vi "VIH Dialog - Enum Values.vi"(8 "VI Path":path, 9 "Control ID":string, 10 "EnumValDefs in":T6[](array[typedef]), 11 "Project Tree":T1) -> (0 "OK out":bool, 2 "EnumValDefs out":T6[](array[typedef]))   [LabVIEW 2014]
doc: "::: VI Helpeks :::\nCopyright (c) 2000-2026 Konstantin Shifershteyn. All rights reserved."
uses:
  _VIH UI Controls.llb/VIH UI Control - Button - Insert HREF.ctl
  _VIH UI Controls.llb/VIH UI Control - Button - Insert Bold.ctl
  _VIH UI Controls.llb/VIH UI Control - Button - Insert Italic.ctl
  _VIH UI Controls.llb/VIH UI Control - Button - Insert Underline.ctl
  _VIH HelpGen.llb/VIH HelpGen Typedef - Cluster - Enum Value Info.ctl
  VIH Project Tree Typedef - Tree Refnum.ctl
  <vilib>/Utility/miscctls.llb/LVRowAndColumnUnsignedTypeDef.ctl
panel:
  in  "%Sort":bool caption="Sort"
  in  "%Import":bool caption="Import"
  in  "%Insert_<I>":T2 caption="Format as Italic"
  in  "%Insert_<U>":T3 caption="Format as Underline"
  in  "%Insert_<B>":T4 caption="Format as Bold"
  in  "%Insert_HREF":T5 caption="Insert Reference"
  in  "Description":string
  in  "String":string
  in  "Value":ext
  in  "%Cancel":bool caption="Cancel"
  in  "%OK":bool caption="OK"
  in  "%Remove":bool caption="Remove"
  in  "%Add":bool caption="Add"
  in  "Val List":i32[](listbox) caption="Value List"
  # "*) use Context Help for information on the controls"
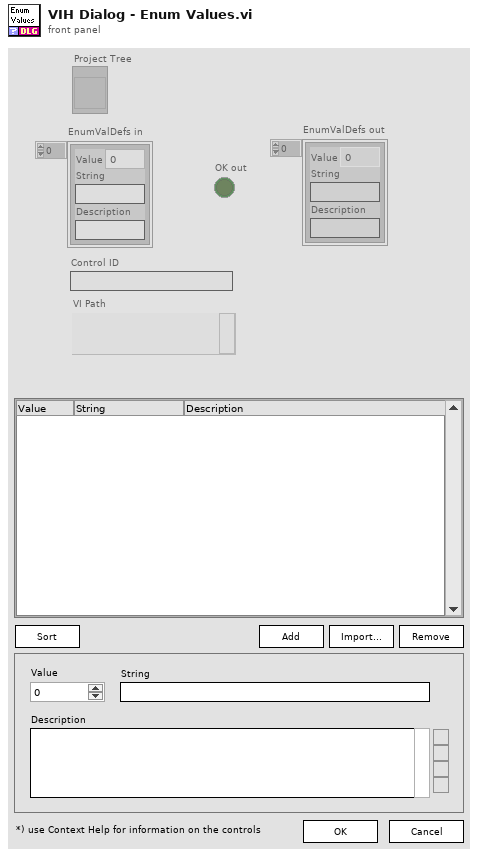
[diagram p1: front panel]
types:
  T1 = typedef "VIH Project Tree Typedef - Tree Refnum.ctl" = refnum<vi>
  T2 = typedef "VIH UI Control - Button - Insert Italic.ctl" = bool
  T3 = typedef "VIH UI Control - Button - Insert Underline.ctl" = bool
  T4 = typedef "VIH UI Control - Button - Insert Bold.ctl" = bool
  T5 = typedef "VIH UI Control - Button - Insert HREF.ctl" = bool
  T6 = typedef "VIH HelpGen Typedef - Cluster - Enum Value Info.ctl" = cluster{"Value":ext, "String":string, "Description":string}
  T7 = typedef "LVRowAndColumnUnsignedTypeDef.ctl" = cluster{"Row":u32, "Column":u32}
  T8 = typedef "lveventtype.ctl" = enum32{"Null", "Timeout", "Annotation Menu Selection", "Annotation Menu Selection?", "App Instance Close", "App Instance Close?", "Autoscale Range Change", "Bookmark Info Change", "Cell Edit", "Cell Edit?", "Cursor Grab", "Cursor Grab?", "Cursor Menu Selection", "Cursor Menu Selection?", "Cursor Move", "Cursor Release", "Data Change", "Direction Change", "Display State Change", "Drag Ended", "Drag Enter", "Drag Leave", "Drag Over", "Drag Source Update", "Drag Starting", "Drag Starting?", "Drop", "Exec State Change", "Key Down", "Key Down?", "Key Repeat", "Key Repeat?", "Key Up", "Listbox Double Click", "Menu Activation?", "Menu Selection (App)", "Menu Selection? (App)", "Menu Selection (User)", "Mouse Down", "Mouse Down?", "Mouse Enter", "Mouse Leave", "Mouse Move", "Mouse Up", "Mouse Wheel", "NI Security User Change (App)", "Pane Size", "Panel Close", "Panel Close?", "Panel Resize", "Plot Attribute Change", "Scale Range Change", "Shortcut Menu Activation?", "Shortcut Menu Selection (App)", "Shortcut Menu Selection? (App)", "Shortcut Menu Selection (User)", "Tree Double Click", "Tree Drag", "Tree Drag?", "Tree Drop", "Tree Drop?", "Tree Item Close", "Tree Item Close?", "Tree Item Open", "Tree Item Open?", "User Event", "Value Change"}
  T9 = enum8{"Enabled", "Disabled", "Disabled and Grayed Out"}
  T10 = typedef "VIH HelpGen Typedef - Cluster - Control Rule.ctl" = cluster{"CtrlID":string, "CustomRule":bool, "DscrMode":T11, "Description":string, "ClusterMembers":T12, "EnumValues":T12, "EnumValDscr":T6[], "CustomName":string}
  T11 = typedef "VIH HelpGen Typedef - Enum - Description Mode.ctl" = enum16{"Default", "Description", "Description1", "Description2", "Custom", "None"}
  T12 = typedef "VIH HelpGen Typedef - Enum - Default,Enable,Disable.ctl" = enum16{"Default", "Enable", "Disable"}
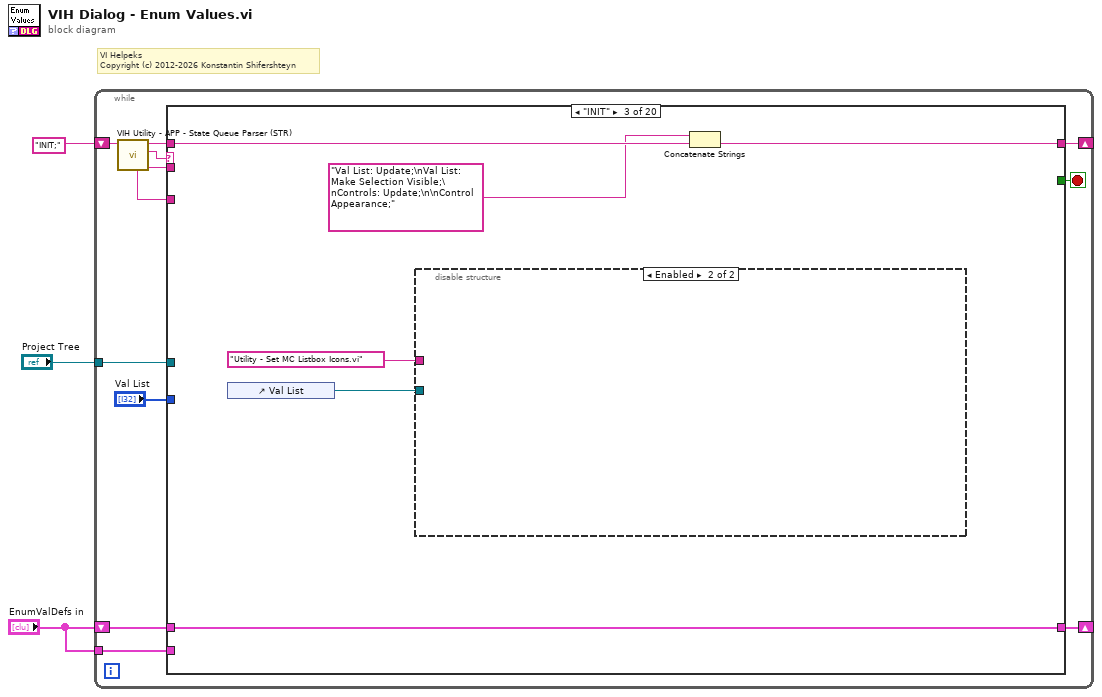
[diagram p0: block diagram]
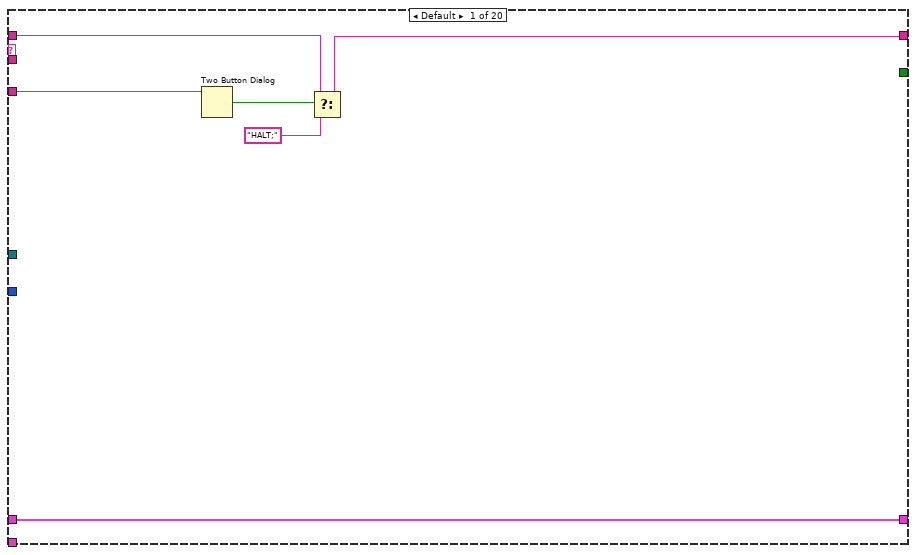
[diagram p2: hidden frame]
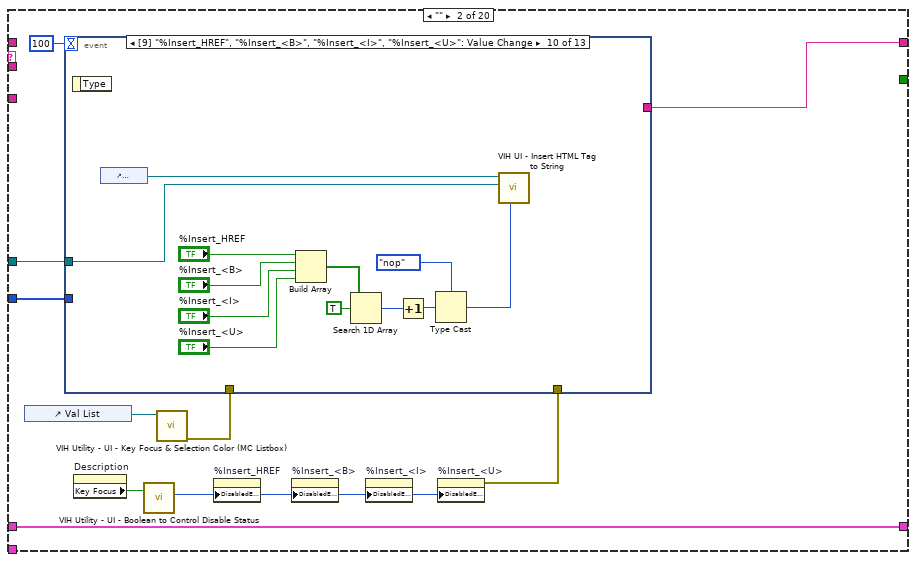
[diagram p3: hidden frame]
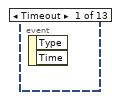
[diagram p4: hidden frame]
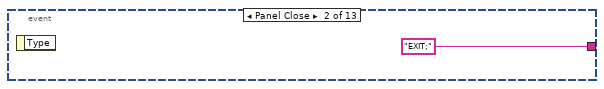
[diagram p5: hidden frame]
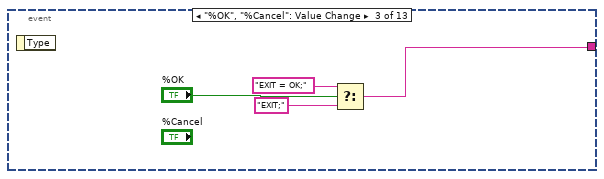
[diagram p6: hidden frame]
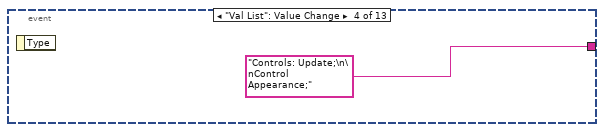
[diagram p7: hidden frame]
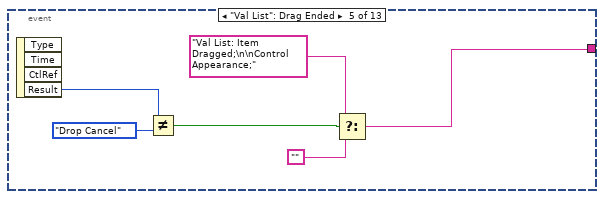
[diagram p8: hidden frame]
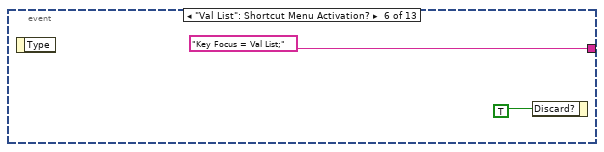
[diagram p9: hidden frame]
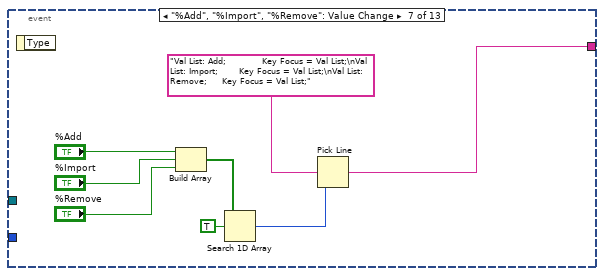
[diagram p10: hidden frame]
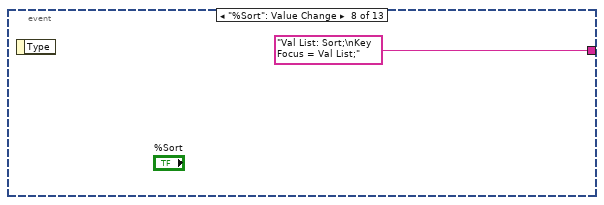
[diagram p11: hidden frame]
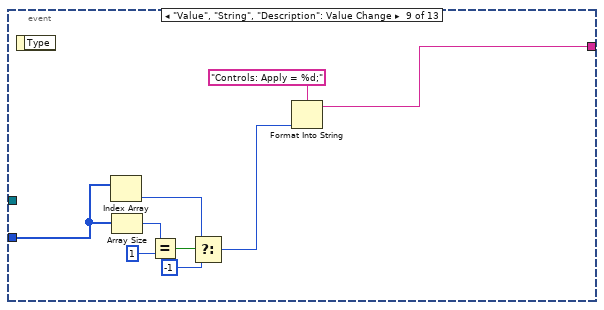
[diagram p12: hidden frame]
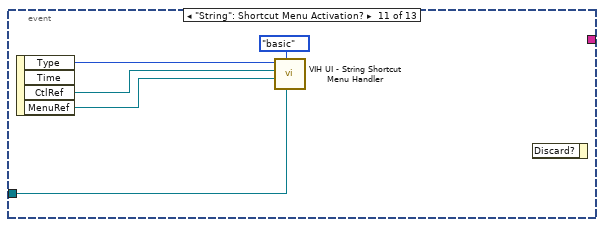
[diagram p13: hidden frame]
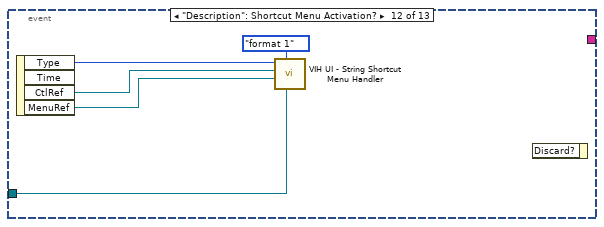
[diagram p14: hidden frame]
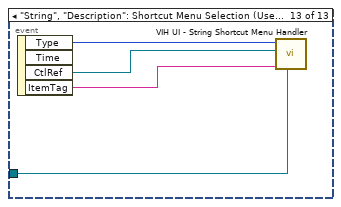
[diagram p15: hidden frame]
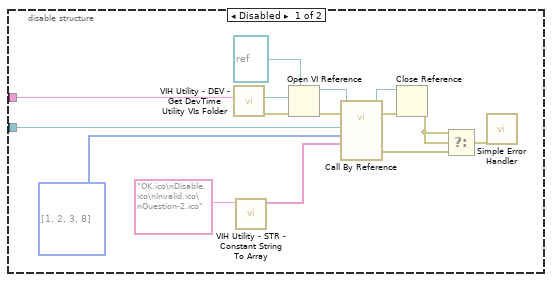
[diagram p16: hidden frame]
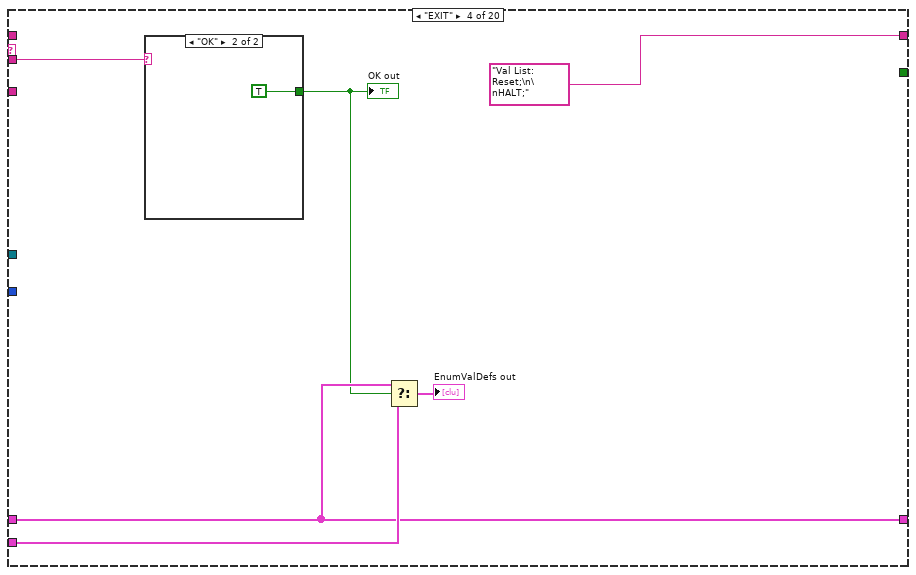
[diagram p17: hidden frame]
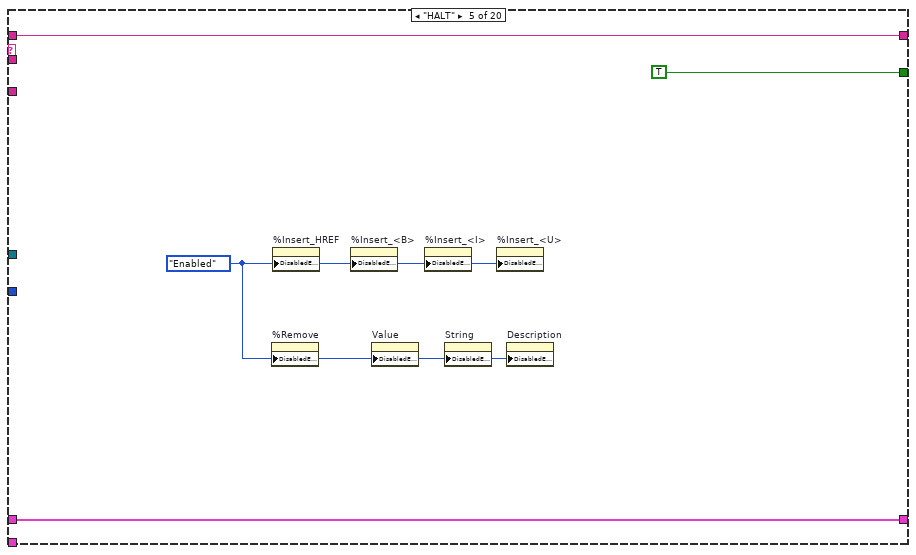
[diagram p19: hidden frame]
diagram:
  # "VI Helpeks\nCopyright (c) 2012-2026 Konstantin Shifershteyn"
  n1 = while {
    shift-right: [w11] -> _
    shift-left: "INIT;" -> [w15]
    shift-right: [w8] -> _
    shift-left: "EnumValDefs in" -> [w9]
    tunnel: "EnumValDefs in" -> [w7]
    tunnel: "Project Tree" -> [w4]
    stop <- w6 stop-if-true
    n2 = call "VIH Utility - APP - State Queue Parser (STR).vi"("input queue"=w15) -> ("state parameters"=w10:string, "state"=w14:string, "remained queue"=w12:string, "complete state specifier"=w13:string)  [unwired: 5 in]
    n3 = case shown="\"INIT\"" w14 {
      tunnel: w13 -> [w21 _ _ _ _ _ _ _ _ _ _ _ _ _ _ _ _ _ _ _]
      tunnel: w12 -> [w19 _ w95 _ w120 w122 w125 w131 w133 w139 w149 w169 w228 w250 w271 w339 w350 w354 w364 w380]
      tunnel: [w18 w30 w94 "Val List: Reset;\n\nHALT;" w120 w122 w125 w131 w133 w139 w148 w169 w228 w249 w270 w338 w345 w354 w364 w374] -> w11
      tunnel: w10 -> [_ _ _ w115 _ _ w124 _ _ _ _ _ _ _ _ _ _ _ _ w377]
      tunnel: w9 -> [w16 w31 w92 w113 w121 w123 w126 w132 w134 _ w144 w165 w229 w230 w267 w325 w347 w355 w361 w379]
      tunnel: [w16 w31 w92 w113 w121 w123 w126 w132 w134 T6[] [] ("EnumValDefs in") w143 w165 w229 w247 w268 w324 w346 w355 w361 w378] -> w8
      tunnel: w7 -> [_ _ _ w114 _ _ _ _ _ _ _ _ _ _ _ _ _ _ _ _]
      tunnel: [_ _ _ _ TRUE _ _ _ _ _ _ _ _ _ _ _ _ _ _ _] -> w6
      tunnel: "Val List" -> [_ w26 _ _ _ _ _ w130 _ _ w142 _ _ w243 _ w326 _ _ w363 _]
      tunnel: w4 -> [_ w22 _ _ _ _ _ _ _ _ _ _ _ _ w262 _ _ _ _ _]
      frame Default {
        n4 = Two Button Dialog(message=w21) -> (T button?=w20:bool)  [unwired: 2 in]
        n5 = Select(t=w19, s=w20, f="HALT;") -> (s? t:f=w18:string)
      }
      frame "" {
        n6 = control-ref of="Val List"() -> (w28:refnum<vi>)
        n7 = property on="Description" class="Str"() -> ("Key Focus"=w25:bool)  [unwired: 2 in, 2 out]
        n8 = call "VIH Utility - UI - Boolean to Control Disable Status.vi"("Status in"=w25) -> ("Control Disable if False"=w23:u8)  [unwired: 3 in, 1 out]
        n9 = call "VIH Utility - UI - Key Focus & Selection Color (MC Listbox).vi"("MCListbox Refnum"=w28) -> ("error out"=w27:errorcluster)  [unwired: 8 in, 2 out]
        n10 = property on="%Insert_HREF" class="Bool"("DisabledEnum"=w23) -> ()  [unwired: 2 in, 2 out]
        n11 = property on="%Insert_<B>" class="Bool"("DisabledEnum"=w23) -> ()  [unwired: 2 in, 2 out]
        n12 = property on="%Insert_<I>" class="Bool"("DisabledEnum"=w23) -> ()  [unwired: 2 in, 2 out]
        n13 = property on="%Insert_<U>" class="Bool"("DisabledEnum"=w23) -> (error out=w24:errorcluster)  [unwired: 2 in, 1 out]
        n14 = event shown="[9] \"%Insert_HREF\", \"%Insert_<B>\", \"%Insert_<I>\", \"%Insert_<U>\": Value Change" {
          selector: _ -> [_ _ _ _ _ _ _ _ _ _ _ _ _]
          dyn-events: _ -> [_ _ _ _ _ _ _ _ _ _ _ _ _]
          timeout: 100 -> [_ _ _ _ _ _ _ _ _ _ _ _ _]
          tunnel: [_ "EXIT;" w35 "Controls: Update;\n\nControl Appearance;" w38 "Key Focus = Val List;" w47 "Val List: Sort;\nKey Focus = Val List;" ("string") w62 _ _ _ _] -> w30
          tunnel: w27 -> [_ _ _ _ _ _ _ _ _ _ _ _ _]
          tunnel: w26 -> [_ _ _ _ _ _ _ _ w58 _ _ _ _]
          tunnel: w24 -> [_ _ _ _ _ _ _ _ _ _ _ _ _]
          tunnel: w22 -> [_ _ _ _ _ _ _ _ _ w68 w76 w81 w87]
          event Timeout {
            n15 = event-data() -> ()  [unwired: 1 in, 2 out]
          }
          event Panel Close {
            n16 = event-data() -> ()  [unwired: 1 in, 1 out]
          }
          event "%OK", "%Cancel": Value Change {
            n17 = event-data() -> ()  [unwired: 1 in, 1 out]
            n18 = Select(t="EXIT = OK;", s="%OK", f="EXIT;") -> (s? t:f=w35:string)
          }
          event "Val List": Value Change {
            n19 = event-data() -> ()  [unwired: 1 in, 1 out]
          }
          event "Val List": Drag Ended {
            n20 = event-data() -> ("Result"=w43:enum16{"Drop Cancel", "Drop Move", "Drop Copy"})  [unwired: 1 in, 3 out]
            n21 = Not Equal?(x=w43, y=enum16{"Drop Cancel", "Drop Move", "Drop Copy"}."Drop Cancel") -> (x != y?=w41:bool)
            n22 = Select(t="Val List: Item Dragged;\n\nControl Appearance;", s=w41, f="") -> (s? t:f=w38:string)
          }
          event "Val List": Shortcut Menu Activation? {
            n23 = event-data() -> ()  [unwired: 1 in, 1 out]
            n24 = event-data("Discard?"=TRUE) -> ()  [unwired: 1 in, 1 out]
          }
          event "%Add", "%Import", "%Remove": Value Change {
            n25 = event-data() -> ()  [unwired: 1 in, 1 out]
            n26 = Build Array("%Add", "%Import", "%Remove") -> (w53:bool[])
            n27 = Search 1D Array(1D array=w53, element=TRUE) -> (index of element=w51:i32)  [unwired: 1 in]
            n28 = Pick Line(multi-line string="Val List: Add;            Key Focus = Val List;\nVal List: Import;       Key Focus = Val List;\nVal List: Remove;     Key Focus = Val List;" ("string"), line index=w51) -> (output string=w47:string)  [unwired: 1 in]
          }
          event "%Sort": Value Change {
            n29 = event-data() -> ()  [unwired: 1 in, 1 out]
          }
          event "Value", "String", "Description": Value Change {
            n30 = event-data() -> ()  [unwired: 1 in, 1 out]
            n31 = Index Array(array=w58) -> (element=w57:i32)  [unwired: 1 in]
            n32 = Array Size(array=w58) -> (size(s)=w61:i32)
            n33 = Equal?(x=w61, y=1) -> (x = y?=w59:bool)
            n34 = Select(t=w57, s=w59, f=-1) -> (s? t:f=w55:i32)
            n35 = Format Into String(format string="Controls: Apply = %d;", w55) -> (resulting string=w62:string)  [unwired: 2 in, 1 out]
          }
          event Value Change {
            n36 = event-data() -> ()  [unwired: 1 in, 1 out]
            n37 = control-ref of="Description"() -> (w69:refnum<vi>)
            n38 = Build Array("%Insert_HREF", "%Insert_<B>", "%Insert_<I>", "%Insert_<U>") -> (w70:T3[])
            n39 = Search 1D Array(1D array=w70, element=TRUE) -> (index of element=w72:i32)  [unwired: 1 in]
            n40 = Increment(x=w72) -> (x+1=w73:i32)
            n41 = Type Cast(type=enum32{"nop", "<a>", "<b>", "<i>", "<u>"}."nop" ("cmd"), x=w73) -> (*(type *) &x=w75:enum32{"nop", "<a>", "<b>", "<i>", "<u>"})
            n42 = call "VIH UI - Insert HTML Tag to String.vi"("cmd"=w75, "Project Tree"=w68, "Str Refnum"=w69) -> ()  [unwired: 8 in, 1 out]
          }
          event "String": Shortcut Menu Activation? {
            n43 = event-data() -> ("Type"=w80:T8, "CtlRef"=w79:refnum<vi>, "MenuRef"=w78:refnum<k9>)  [unwired: 1 in, 1 out]
            n44 = call "VIH UI - String Shortcut Menu Handler.vi"("Project Tree"=w76, "mode"=enum16{"basic", "format 1", "format 2"}."basic", "menu"=w78, "Str Refnum"=w79, "Type"=w80) -> ()  [unwired: 7 in]
            n45 = event-data() -> ()  [unwired: 2 in, 1 out]
          }
          event "Description": Shortcut Menu Activation? {
            n46 = event-data() -> ("Type"=w85:T8, "CtlRef"=w84:refnum<vi>, "MenuRef"=w83:refnum<k9>)  [unwired: 1 in, 1 out]
            n47 = call "VIH UI - String Shortcut Menu Handler.vi"("Project Tree"=w81, "mode"=enum16{"basic", "format 1", "format 2"}."format 1", "menu"=w83, "Str Refnum"=w84, "Type"=w85) -> ()  [unwired: 7 in]
            n48 = event-data() -> ()  [unwired: 2 in, 1 out]
          }
          event "String", "Description": Shortcut Menu Selection (User) {
            n49 = event-data() -> ("Type"=w89:T8, "CtlRef"=w88:refnum<vi>, "ItemTag"=w86:string)  [unwired: 1 in, 1 out]
            n50 = call "VIH UI - String Shortcut Menu Handler.vi"("Project Tree"=w87, "Menu tag"=w86, "Str Refnum"=w88, "Type"=w89) -> ()  [unwired: 8 in]
          }
        }
      }
      frame "INIT" {
        n51 = control-ref of="Val List"() -> (w91:refnum<vi>)
        n52 = disable-structure shown="Enabled" {
          disable-tunnel: w91 -> [w102 _]
          disable-tunnel: "Utility - Set MC Listbox Icons.vi" ("Utility VI Name") -> [w99 _]
          frame Disabled {
            n53 = call "VIH Utility - DEV - Get DevTime Utility VIs Folder.vi"("Utility VI Name"=w99) -> ("error out"=w106:errorcluster, "Utility VIs Path"=w105:path)  [unwired: 8 in, 1 out]
            n54 = call "VIH Utility - STR - Constant String To Array.vi"("String in"="OK.ico\nDisable.ico\nInvalid.ico\nQuestion-2.ico") -> ("Array out"=w100:string[])  [unwired: 10 in]
            n55 = Open VI Reference(type specifier VI Refnum (for type only)=refnum<vi> refnum, vi path=w105, error in (no error)=w106) -> (vi reference=w108:refnum<vi>, error out=w109:errorcluster)  [unwired: 3 in]
            n56 = call-by-ref "?"(reference=w108, error in=w109, "Icon Filenames"=w100, "Symbol Indices"=i32[] [1, 2, 3, 8], "MCListbox Refnum"=w102) -> (reference out=w103:refnum<vi>, error out=w104:errorcluster, 0:"error out"=w97:errorcluster)  [unwired: 8 in]
            n57 = Close Reference(reference=w103, error in (no error)=w104) -> (error out=w98:errorcluster)
            n58 = Select(t=w98, s=w98, f=w97) -> (s? t:f=w96:errorcluster)
            n59 = call <vilib>:"Simple Error Handler.vi"("error in (no error)"=w96) -> ()  [unwired: 4 in, 5 out]
          }
          frame Enabled {
          }
        }
        n60 = Concatenate Strings("Val List: Update;\nVal List: Make Selection Visible;\nControls: Update;\n\nControl Appearance;", w95) -> (w94:string)
      }
      frame "EXIT" {
        n61 = case shown="\"OK\"" w115 {
          tunnel: [_ TRUE] -> w112
          frame Default {
          }
          frame "OK" {
          }
        }
        "OK out" <- w112
        n62 = Select(t=w113, s=w112, f=w114) -> (s? t:f=→"EnumValDefs out":T6[])
      }
      frame "HALT" {
        w118 = T9."Enabled" ("Disabled")
        n63 = property on="%Remove" class="Bool"("DisabledEnum"=w118) -> ()  [unwired: 2 in, 2 out]
        n64 = property on="%Insert_HREF" class="Bool"("DisabledEnum"=w118) -> ()  [unwired: 2 in, 2 out]
        n65 = property on="%Insert_<B>" class="Bool"("DisabledEnum"=w118) -> ()  [unwired: 2 in, 2 out]
        n66 = property on="Value" class="DigNum (strict)"("DisabledEnum"=w118) -> ()  [unwired: 2 in, 2 out]
        n67 = property on="%Insert_<I>" class="Bool"("DisabledEnum"=w118) -> ()  [unwired: 2 in, 2 out]
        n68 = property on="String" class="Str"("DisabledEnum"=w118) -> ()  [unwired: 2 in, 2 out]
        n69 = property on="%Insert_<U>" class="Bool"("DisabledEnum"=w118) -> ()  [unwired: 2 in, 2 out]
        n70 = property on="Description" class="Str"("DisabledEnum"=w118) -> ()  [unwired: 2 in, 2 out]
      }
      frame "--------------------------------- 1" {
      }
      frame "Key Focus" {
        n71 = case shown="\"Val List\"" w124 {
          frame Default {
          }
          frame "Val List" {
            n72 = property on="Val List" class="MCListbox (strict)"("Key Focus"=TRUE) -> ()  [unwired: 2 in, 2 out]
          }
        }
      }
      frame "Control Appearance" {
        n73 = Empty Array?(array=w130) -> (empty?=w129:bool)
        n74 = call "VIH Utility - UI - Boolean to Control Disable Status.vi"("Status in"=w129) -> ("Control Disable if True"=w128:u8)  [unwired: 3 in, 1 out]
        n75 = property on="%Remove" class="Bool"("DisabledEnum"=w128) -> ()  [unwired: 2 in, 2 out]
      }
      frame "--------------------------------- 2" {
      }
      frame "Val List: Reset" {
        w137 = i32[] [] ("Item Symbols")
        n76 = property on="Val List" class="MCListbox (strict)"("TopLeft"=T7 {"Row"=0, "Column"=0} ("Top Left Visible Cell"), "Value"=w137, "ItemNames"=string[][] [] ("Item Names"), "ItemSyms"=w137) -> ()  [unwired: 2 in, 2 out]
      }
      frame "Val List: Sort" {
        n77 = for {
          tunnel: w144 -> [w162] mode=indexing
          tunnel: [w159] -> w146 mode=indexing
          i -> [w157]
          n78 = Unbundle(w162) -> ("Value"=w161:ext, "String"=w160:string)  [unwired: 1 out]
          n79 = To Lower Case(string=w160) -> (all lower case string=w158:string)
          n80 = Bundle("Value"=w161, w158, w157) -> (w159:cluster{"Value":ext, string, i32})  [unwired: 1 in]
        }
        n81 = Sort 1D Array(array=w146) -> (sorted array=w145:cluster{"Value":ext, string, i32}[])
        n82 = for {
          tunnel: w145 -> [w156] mode=indexing
          tunnel: w144 -> [w155]
          tunnel: [w154] -> w143 mode=indexing
          tunnel: [w153] -> w141 mode=indexing
          n83 = Unbundle(w156) -> (w153:i32)  [unwired: 2 out]
          n84 = Index Array(array=w155, index=w153) -> (element=w154:T6)
        }
        n85 = for {
          tunnel: w142 -> [w152] mode=indexing
          tunnel: w141 -> [w151]
          tunnel: [w150] -> w140 mode=indexing
          n86 = Search 1D Array(1D array=w151, element=w152) -> (index of element=w150:i32)  [unwired: 1 in]
        }
        n87 = Concatenate Strings("Val List: Update;\nVal List: Make Selection Visible;\n\nControls: Update;\n\nControl Appearance;" ("string"), w149) -> (w148:string)
        n88 = local write "Val List"(w140) -> ()
      }
      frame "Val List: Update" {
        n89 = for {
          tunnel: w165 -> [w171] mode=indexing
          tunnel: [w170] -> w164 mode=indexing
          n90 = Unbundle By Name(w171) -> ("Value"=w170:ext)
        }
        n91 = for {
          tunnel: w165 -> [w196] mode=indexing
          tunnel: [w187] -> w168 mode=indexing
          tunnel: w164 -> [w180]
          tunnel: [w173] -> w163 mode=indexing
          i -> [w177]
          w190 = 40 ("y")
          n92 = Unbundle By Name(w196) -> ("Value"=w179:ext, "String"=w189:string, "Description"=w182:string)
          n93 = call <vilib>:"Trim Whitespace.vi"("string"=w182) -> ("trimmed string"=w181:string)  [unwired: 1 in]
          n94 = Search/Split String(string=w181, search string/char (-)="\n") -> (substring before match=w191:string, offset of match=w186:i32)  [unwired: 1 in, 1 out]
          n95 = for {
            N: 2 -> [_]
            tunnel: w180 -> [w207]
            tunnel: w179 -> [w206]
            tunnel: w177 -> [w205]
            tunnel: [w200] -> w176
            shift-right: [w197] -> _
            shift-left: 0 -> [w202]
            stop <- w201 stop-if-true
            n96 = Search 1D Array(1D array=w207, element=w206, start index (0)=w202) -> (index of element=w198:i32)
            n97 = Greater Or Equal To 0?(x=w198) -> (x >= 0?=w204:bool)
            n98 = Not Equal?(x=w198, y=w205) -> (x != y?=w203:bool)
            n99 = Less Than 0?(x=w198) -> (x < 0?=w199:bool)
            n100 = Increment(x=w198) -> (x+1=w197:i32)
            n101 = And(x=w204, y=w203) -> (x .and. y?=w200:bool)
            n102 = Or(x=w200, y=w199) -> (x .or. y?=w201:bool)
          }
          n103 = String Length(string=w191) -> (length=w193:i32)
          n104 = Greater?(x=w193, y=w190) -> (0:w192:bool)
          n105 = case shown="True" w192 {
            tunnel: w191 -> [w214 w220]
            tunnel: w190 -> [_ w219]
            tunnel: [w214 w216] -> w185
            tunnel: w186 -> [w213 _]
            tunnel: [w212 TRUE] -> w183
            frame False {
              n106 = Greater Or Equal To 0?(x=w213) -> (x >= 0?=w212:bool)
            }
            frame True {
              n107 = Subtract(x=w219, y=3) -> (x-y=w217:i32)
              n108 = String Subset(string=w220, length (rest)=w217) -> (substring=w216:string)  [unwired: 1 in]
            }
          }
          n109 = case shown="True" w183 {
            tunnel: w185 -> [w208 w210]
            tunnel: [w208 w209] -> w184
            frame False {
            }
            frame True {
              n110 = Concatenate Strings(w210, "...") -> (w209:string)
            }
          }
          n111 = Format Into String(format string="%.;%#f", w179) -> (resulting string=w188:string)  [unwired: 2 in, 1 out]
          n112 = Select(t=8, s=w176, f=0) -> (s? t:f=w173:i32)
          n113 = Build Array(w188, w189, w184) -> (w187:string[])
        }
        n114 = call "VIH Utility - UI - Drag and Drop Supporter (w Symbol Indices).vi"("Cmd"=enum16{"make symbols", "test D'n'D"}."make symbols", "Item Symbols"=w163) -> ("Item Symbols out"=w167:i32[])  [unwired: 7 in, 2 out]
        n115 = property on="Val List" class="MCListbox (strict)"("ItemNames"=w168, "ItemSyms"=w167) -> ()  [unwired: 2 in, 2 out]
      }
      frame "Val List: Make Selection Visible" {
        n116 = control-ref of="Val List"() -> (w223:refnum<vi>)
        n117 = property class="MCListbox (strict)"(reference=w223) -> (reference out=w225:refnum<vi>, "Value"=w222:i32[])  [unwired: 1 in, 1 out]
        n118 = Array Max & Min(array=w222) -> (min value=w221:i32)  [unwired: 3 out]
        n119 = Empty Array?(array=w222) -> (empty?=w226:bool)
        n120 = Select(t=-1, s=w226, f=w221) -> (s? t:f=w224:i32)
        n121 = call "VIH Utility - UI - Make Row Visible (MC Listbox).vi"("Row"=w224, "MC Listbox Refnum"=w225) -> ()  [unwired: 8 in, 2 out]
      }
      frame "Val List: Add" {
        n122 = Array Size(array=w243) -> (size(s)=w246:i32)
        n123 = Array Max & Min(array=w243) -> (max value=w244:i32)  [unwired: 3 out]
        n124 = Less Or Equal To 0?(x=w246) -> (x <= 0?=w245:bool)
        n125 = Select(t=-1, s=w245, f=w244) -> (s? t:f=w236:i32)
        n126 = Empty Array?(array=w230) -> (empty?=w231:bool)
        n127 = Increment(x=w236) -> (x+1=w241:i32)
        n128 = case shown="False" w231 {
          tunnel: w230 -> [w255 _]
          tunnel: [w252 _] -> w232
          frame False {
            n129 = for {
              tunnel: w255 -> [w257] mode=indexing
              tunnel: [w256] -> w254 mode=indexing
              n130 = Unbundle By Name(w257) -> ("Value"=w256:ext)
            }
            n131 = Array Max & Min(array=w254) -> (max value=w253:ext)  [unwired: 3 out]
            n132 = Round Toward -Infinity(1:w253) -> (0:w251:ext)
            n133 = Increment(x=w251) -> (x+1=w252:ext)
          }
          frame True {
          }
        }
        n134 = Array Size(array=w230) -> (size(s)=w240:i32)
        n135 = Index Array(array=w230, index=-1) -> (element=w234:T6)
        n136 = In Range and Coerce(upper limit=w240, x=w241, lower limit=0) -> (coerced(x)=w238:i32)  [unwired: 1 out]
        n137 = Bundle By Name(cluster=w234, "Value"=w232) -> (w233:T6)
        n138 = Build Array(w238) -> (w237:i32[])
        n139 = Concatenate Strings("Val List: Update;\nVal List: Make Selection Visible;\n\nControls: Update;\n\nControl Appearance;" ("string"), w250) -> (w249:string)
        n140 = local write "Val List"(w237) -> ()
        n141 = Insert Into Array(array=w230, index=w238, new element=w233) -> (w247:T6[])
      }
      frame "Val List: Import" {
        n142 = Empty String/Path?(string/path="VI Path") -> (empty?=w265:bool)
        n143 = case shown="True" w265 {
          tunnel: [w318 w322] -> w264
          tunnel: [TRUE w321] -> w263
          tunnel: "VI Path" -> [w318 _]
          tunnel: w262 -> [_ w320]
          frame False {
          }
          frame True {
            n144 = call "VIH Dialog - Project File List.vi"("File set (All)"=enum32{"ALL", "conpane", "invalid"}."conpane", "Project Tree"=w320) -> ("OK out"=w321:bool, "File Path"=w322:path)  [unwired: 7 in, 1 out]
          }
        }
        n145 = Build Array("Control ID") -> (w258:string[])
        n146 = case shown="True" w263 {
          selector: w263 -> [w309 _]
          tunnel: w264 -> [_ w314]
          tunnel: [w309 w313] -> w260
          tunnel: [_ w312] -> w261
          tunnel: w258 -> [_ w310]
          frame False {
          }
          frame True {
            n147 = call "VIH Dialog - VI Terminals.vi"("mode (normal)"=enum16{"normal", "Enum sel"}."Enum sel", "Ctrl IDs in"=w310, "VI Path"=w314) -> ("OK out"=w313:bool, "Ctrl Rules"=w315:T10[])  [unwired: 5 in, 2 out]
            n148 = Index Array(array=w315) -> (element=w316:T10)  [unwired: 1 in]
            n149 = Unbundle By Name(w316) -> ("EnumValDscr"=w312:T6[])
          }
        }
        n150 = case shown="True" w260 {
          tunnel: [w272 w282] -> w268
          tunnel: w267 -> [w272 w281]
          tunnel: w261 -> [_ w279]
          frame False {
          }
          frame True {
            n151 = for {
              tunnel: w281 -> [w286] mode=indexing
              tunnel: [w283] -> w280 mode=indexing
              n152 = Unbundle(w286) -> ("Value"=w285:ext, "String"=w284:string)  [unwired: 1 out]
              n153 = Bundle("Value"=w285, "String"=w284) -> (w283:cluster{"Value":ext, "String":string})  [unwired: 1 in]
            }
            n154 = Array Size(array=w281) -> (size(s)=w273:i32)
            n155 = for {
              tunnel: w279 -> [w289] mode=indexing
              tunnel: w280 -> [w296]
              shift-right: [w292] -> w277
              shift-left: w279 -> [w293]
              shift-right: [w290] -> w276
              shift-left: 0 -> [w291]
              tunnel: [w288] -> w274 mode=indexing
              tunnel: w273 -> [w287]
              n156 = Unbundle(w289) -> ("Value"=w298:ext, "String"=w297:string)  [unwired: 1 out]
              n157 = Bundle("Value"=w298, "String"=w297) -> (w295:cluster{"Value":ext, "String":string})  [unwired: 1 in]
              n158 = Search 1D Array(1D array=w296, element=w295) -> (index of element=w294:i32)  [unwired: 1 in]
              n159 = case shown="..-1" w294 {
                selector: w294 -> [_ w306]
                tunnel: w293 -> [w305 w308]
                tunnel: [w304 w308] -> w292
                tunnel: w291 -> [w301 w307]
                tunnel: [w303 w307] -> w290
                tunnel: w289 -> [w302 _]
                tunnel: [w299 w306] -> w288
                tunnel: w287 -> [w300 _]
                frame ..-1 {
                  n160 = Add(x=w300, y=w301) -> (x+y=w299:i32)
                  n161 = Replace Array Subset(array=w305, new element=w302, index=w301) -> (w304:T6[])
                  n162 = Increment(x=w301) -> (x+1=w303:i32)
                }
                frame 0.. {
                }
              }
            }
            n163 = local write "Val List"(w274) -> ()
            n164 = Reshape Array(w277, w276) -> (w275:T6[])
            n165 = Insert Into Array(array=w281, index=w273, new element=w275) -> (w282:T6[])
          }
        }
        n166 = Concatenate Strings("Val List: Update;\nVal List: Make Selection Visible;\n\nControls: Update;\n\nControl Appearance;" ("string"), w271) -> (w270:string)
      }
      frame "Val List: Remove" {
        n167 = Sort 1D Array(array=w326) -> (sorted array=w336:i32[])
        n168 = Reverse 1D Array(array=w336) -> (reversed array=w327:i32[])
        n169 = for {
          tunnel: w327 -> [w340] mode=indexing
          shift-right: [w342] -> w324
          shift-left: w325 -> [w341]
          n170 = Delete From Array(array=w341, index=w340) -> (array with subset deleted=w342:T6[])  [unwired: 1 in, 1 out]
        }
        n171 = Index Array(array=w336) -> (element=w328:i32)  [unwired: 1 in]
        n172 = Array Size(array=w324) -> (size(s)=w330:i32)
        n173 = Decrement(x=w330) -> (x-1=w335:i32)
        n174 = In Range and Coerce(upper limit=w335, x=w328, lower limit=0) -> (coerced(x)=w332:i32)  [unwired: 1 out]
        n175 = Less Than 0?(x=w335) -> (x < 0?=w331:bool)
        n176 = Build Array(w332) -> (w333:i32[])
        n177 = Select(t=i32[] [] ("CSS List"), s=w331, f=w333) -> (s? t:f=w323:i32[])
        n178 = local write "Val List"(w323) -> ()
        n179 = Concatenate Strings("Val List: Update;\nVal List: Make Selection Visible;\n\nControls: Update;\n\nControl Appearance;" ("string"), w339) -> (w338:string)
      }
      frame "Val List: Item Dragged" {
        n180 = property on="Val List" class="MCListbox (strict)"() -> ("ItemSyms"=w349:i32[])  [unwired: 2 in, 2 out]
        n181 = call "VIH Utility - UI - Drag and Drop Supporter (w Symbol Indices).vi"("Cmd"=enum16{"make symbols", "test D'n'D"}."test D'n'D", "Item Symbols"=w349) -> ("indices"=w348:i32[])  [unwired: 7 in, 2 out]
        n182 = for {
          tunnel: w348 -> [w353] mode=indexing
          tunnel: w347 -> [w352]
          tunnel: [w351] -> w346 mode=indexing
          n183 = Index Array(array=w352, index=w353) -> (element=w351:T6)
        }
        n184 = Concatenate Strings("Val List: Update;\n\nControls: Update;\n\nControl Appearance;" ("string"), w350) -> (w345:string)
      }
      frame "--------------------------------- 3" {
      }
      frame "Controls: Update" {
        n185 = Index Array(array=w363) -> (element=w360:i32)  [unwired: 1 in]
        n186 = Array Size(array=w363) -> (size(s)=w362:i32)
        n187 = case shown="1" w362 {
          tunnel: w361 -> [_ w372]
          tunnel: w360 -> [_ w371]
          tunnel: [u8 2 _] -> w359
          tunnel: [_ w369] -> w358
          tunnel: [_ w368] -> w357
          tunnel: [_ w366] -> w356
          frame Default {
          }
          frame 1 {
            n188 = Index Array(array=w372, index=w371) -> (element=w370:T6)
            n189 = Unbundle By Name(w370) -> ("Value"=w369:ext, "String"=w368:string, "Description"=w367:string)
            n190 = call <vilib>:"Trim Whitespace.vi"("string"=w367) -> ("trimmed string"=w366:string)  [unwired: 1 in]
          }
        }
        n191 = property on="Value" class="DigNum (strict)"("DisabledEnum"=w359, "Value"=w358) -> ()  [unwired: 2 in, 2 out]
        n192 = property on="String" class="Str"("DisabledEnum"=w359, "Value"=w357) -> ()  [unwired: 2 in, 2 out]
        n193 = property on="Description" class="Str"("DisabledEnum"=w359, "Value"=w356) -> ()  [unwired: 2 in, 2 out]
      }
      frame "Controls: Apply" {
        n194 = Decimal String To Number(string=w377, default (0L)=-1 ("default (0 I32)")) -> (number=w375:i32)  [unwired: 1 in, 1 out]
        n195 = in-place {
          n196 = in-place-array #1(w379, w375) -> (w386:T6)
          n197 = call <vilib>:"Trim Whitespace.vi"("string"="Description") -> ("trimmed string"=w381:string)  [unwired: 1 in]
          n198 = Bundle By Name(cluster=w386, "Value"="Value", "String"="String", "Description"=w381) -> (w385:T6)
          n199 = in-place-array #1(w385) -> (w378:T6[])  [unwired: 1 out]
        }
        n200 = Concatenate Strings("Val List: Update;\n\nControls: Update;\n\nControl Appearance;", w380) -> (w374:string)
      }
    }
  }
